vi "Teleop.vi"(10 "Match Info":T1={"Autonomous Elapsed Seconds"=0.0, "TeleOp Elapsed Seconds"=0.0, "Disabled Elapsed Seconds"=0.0, "Visited Autonomous"=FALSE, "Visited TeleOp"=FALSE, "Visited Disabled"=FALSE, "Autonomous Settings"={"Autonomous Style"=enum."Independent", "VI Refnum"=refnum}}, 11 "Call Context":T2) -> ()   [LabVIEW 2016]
doc: "This VI is called for each TeleOp packet received from the DS where the robot is not disabled. It is often used to read from the joysticks and update I/O or to update setpoints for timed control loops. It should complete and return within 20 milliseconds or it may miss DS packets."
uses:
  <vilib>/Rock Robotics/WPI/DriverStation/WPI_DriverStationDerivedRobotMode.ctl
  <vilib>/Rock Robotics/WPI/DriverStation/WPI_DriverStationMatch Info.ctl
  <vilib>/Rock Robotics/WPI/Solenoid/WPI_SolenoidValue.ctl
  <vilib>/Rock Robotics/WPI/Relay/WPI_RelayValue.ctl
  <vilib>/Rock Robotics/WPI/ThirdParty/CanMotor/TalonSRX/WPI_CANTalonSRX_BrakeOverride.ctl
  <vilib>/Rock Robotics/WPI/Utilities/WPI_GetSetVariantRefNum.vi
  <vilib>/Rock Robotics/Network Tables/NT Write Boolean Array.vi
  <vilib>/Rock Robotics/Network Tables/NT Write Numeric Array.vi
  <vilib>/Rock Robotics/Network Tables/NT Read Boolean.vi
  <vilib>/Rock Robotics/Network Tables/NT Read Number.vi
  <vilib>/Rock Robotics/WPI/Solenoid/WPI_SolenoidSetEnum.vi
  <vilib>/Rock Robotics/Network Tables/NT Write Boolean.vi
  <vilib>/Rock Robotics/WPI/RobotDrive/WPI_RobotDriveArcadeDrive_Standard(NoSaturation).vi
panel:
  out "Sample Slider 0":dbl(slide) scale=0.0..5.0
  out "Sample Boolean 1":bool
  out "Sample Boolean 0":bool
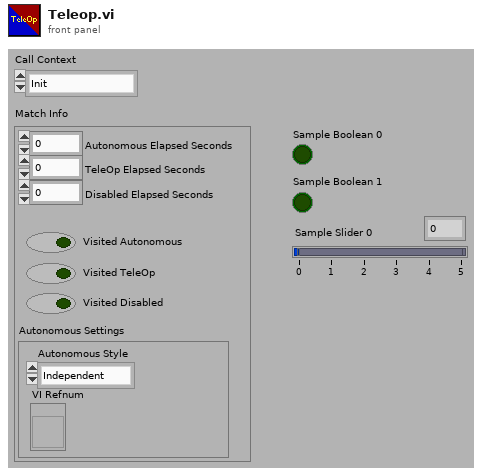
[diagram p1: front panel]
types:
  T1 = typedef "WPI_DriverStationMatch Info.ctl" = cluster{"Autonomous Elapsed Seconds":dbl, "TeleOp Elapsed Seconds":dbl, "Disabled Elapsed Seconds":dbl, "Visited Autonomous":bool, "Visited TeleOp":bool, "Visited Disabled":bool, "Autonomous Settings":cluster{"Autonomous Style":enum16{"Iterative", "Independent"}, "VI Refnum":refnum<vi>}}
  T2 = typedef "WPI_DriverStationDerivedRobotMode.ctl" = enum16{"Init", "Execute", "Stop"}
  T3 = typedef "WPI_CANTalonSRX_BrakeOverride.ctl" = enum8{"No Override", "Override to Coast", "Override to Brake"}
  T4 = typedef "WPI_SolenoidValue.ctl" = enum16{"Off", "On", "Forward", "Reverse"}
  T5 = typedef "WPI_RelayValue.ctl" = enum16{"Off", "On", "Forward", "Reverse"}
  T6 = typedef "WPI_JoystickDevRef.ctl" = cluster{"Device":T7}
  T7 = typedef "WPI_JoystickDeviceEnum.ctl" = enum16{"USB 0", "USB 1", "USB 2", "USB 3", "USB 4", "USB 5"}
  T8 = typedef "WPI_MotorControlDeviceRef.ctl" = cluster{"DeviceStatus":errorcluster, "Type":T9, "PWM":cluster{"PWM Channel":T10, "DeadBand":T11}, "CAN":cluster{"Device Number":u8, "SetOutput VI Ref":variant, "GetOutput VI Ref":variant, "Enable VI Ref":variant, "Disable VI Ref":variant, "Data":variant}, "Invert":bool}
  T9 = typedef "WPI_MotorControlType.ctl" = enum16{"PWM", "CAN"}
  T10 = typedef "FPGA_DIOPWMChannel.ctl" = enum8{"PWM 0", "PWM 1", "PWM 2", "PWM 3", "PWM 4", "PWM 5", "PWM 6", "PWM 7", "PWM 8", "PWM 9", "PWM MXP 0", "PWM MXP 1", "PWM MXP 2", "PWM MXP 3", "PWM MXP 4", "PWM MXP 5", "PWM MXP 6", "PWM MXP 7", "PWM MXP 8", "PWM MXP 9", "Invalid"}
  T11 = typedef "WPI_PWMDeadband.ctl" = cluster{"Name":string, "maxPositivePwm":i32, "minPositivePwm":i32, "centerPwm":i32, "maxNegativePwm":i32, "minNegativePwm":i32, "angularRange":u16}
  T12 = typedef "WPI_RobotDriveDevRef.ctl" = cluster{"DevStatus":errorcluster, "Motors[]":T8[], "Square Inputs":bool, "Max Output":dbl}
  T13 = typedef "WPI_RelayDevRef.ctl" = cluster{"DevStatus":errorcluster, "Relay Channel":T14, "Relay Direction":T15}
  T14 = typedef "FPGA_DIORelayChannel.ctl" = enum8{"Relay 0", "Relay 1", "Relay 2", "Relay 3", "Invalid"}
  T15 = typedef "WPI_RelayDirection.ctl" = enum16{"Both directions", "Forward only", "Reverse only"}
  T16 = typedef "WPI_SolenoidDevRef.ctl" = cluster{"DevStatus":errorcluster, "Pneumatics Control Module":u8, "Forward Solenoid Channel":T17, "Reverse Solenoid Channel":T17}
  T17 = typedef "WPI_SolenoidChannel.ctl" = enum8{"Solenoid 0", "Solenoid 1", "Solenoid 2", "Solenoid 3", "Solenoid 4", "Solenoid 5", "Solenoid 6", "Solenoid 7", "Invalid"}
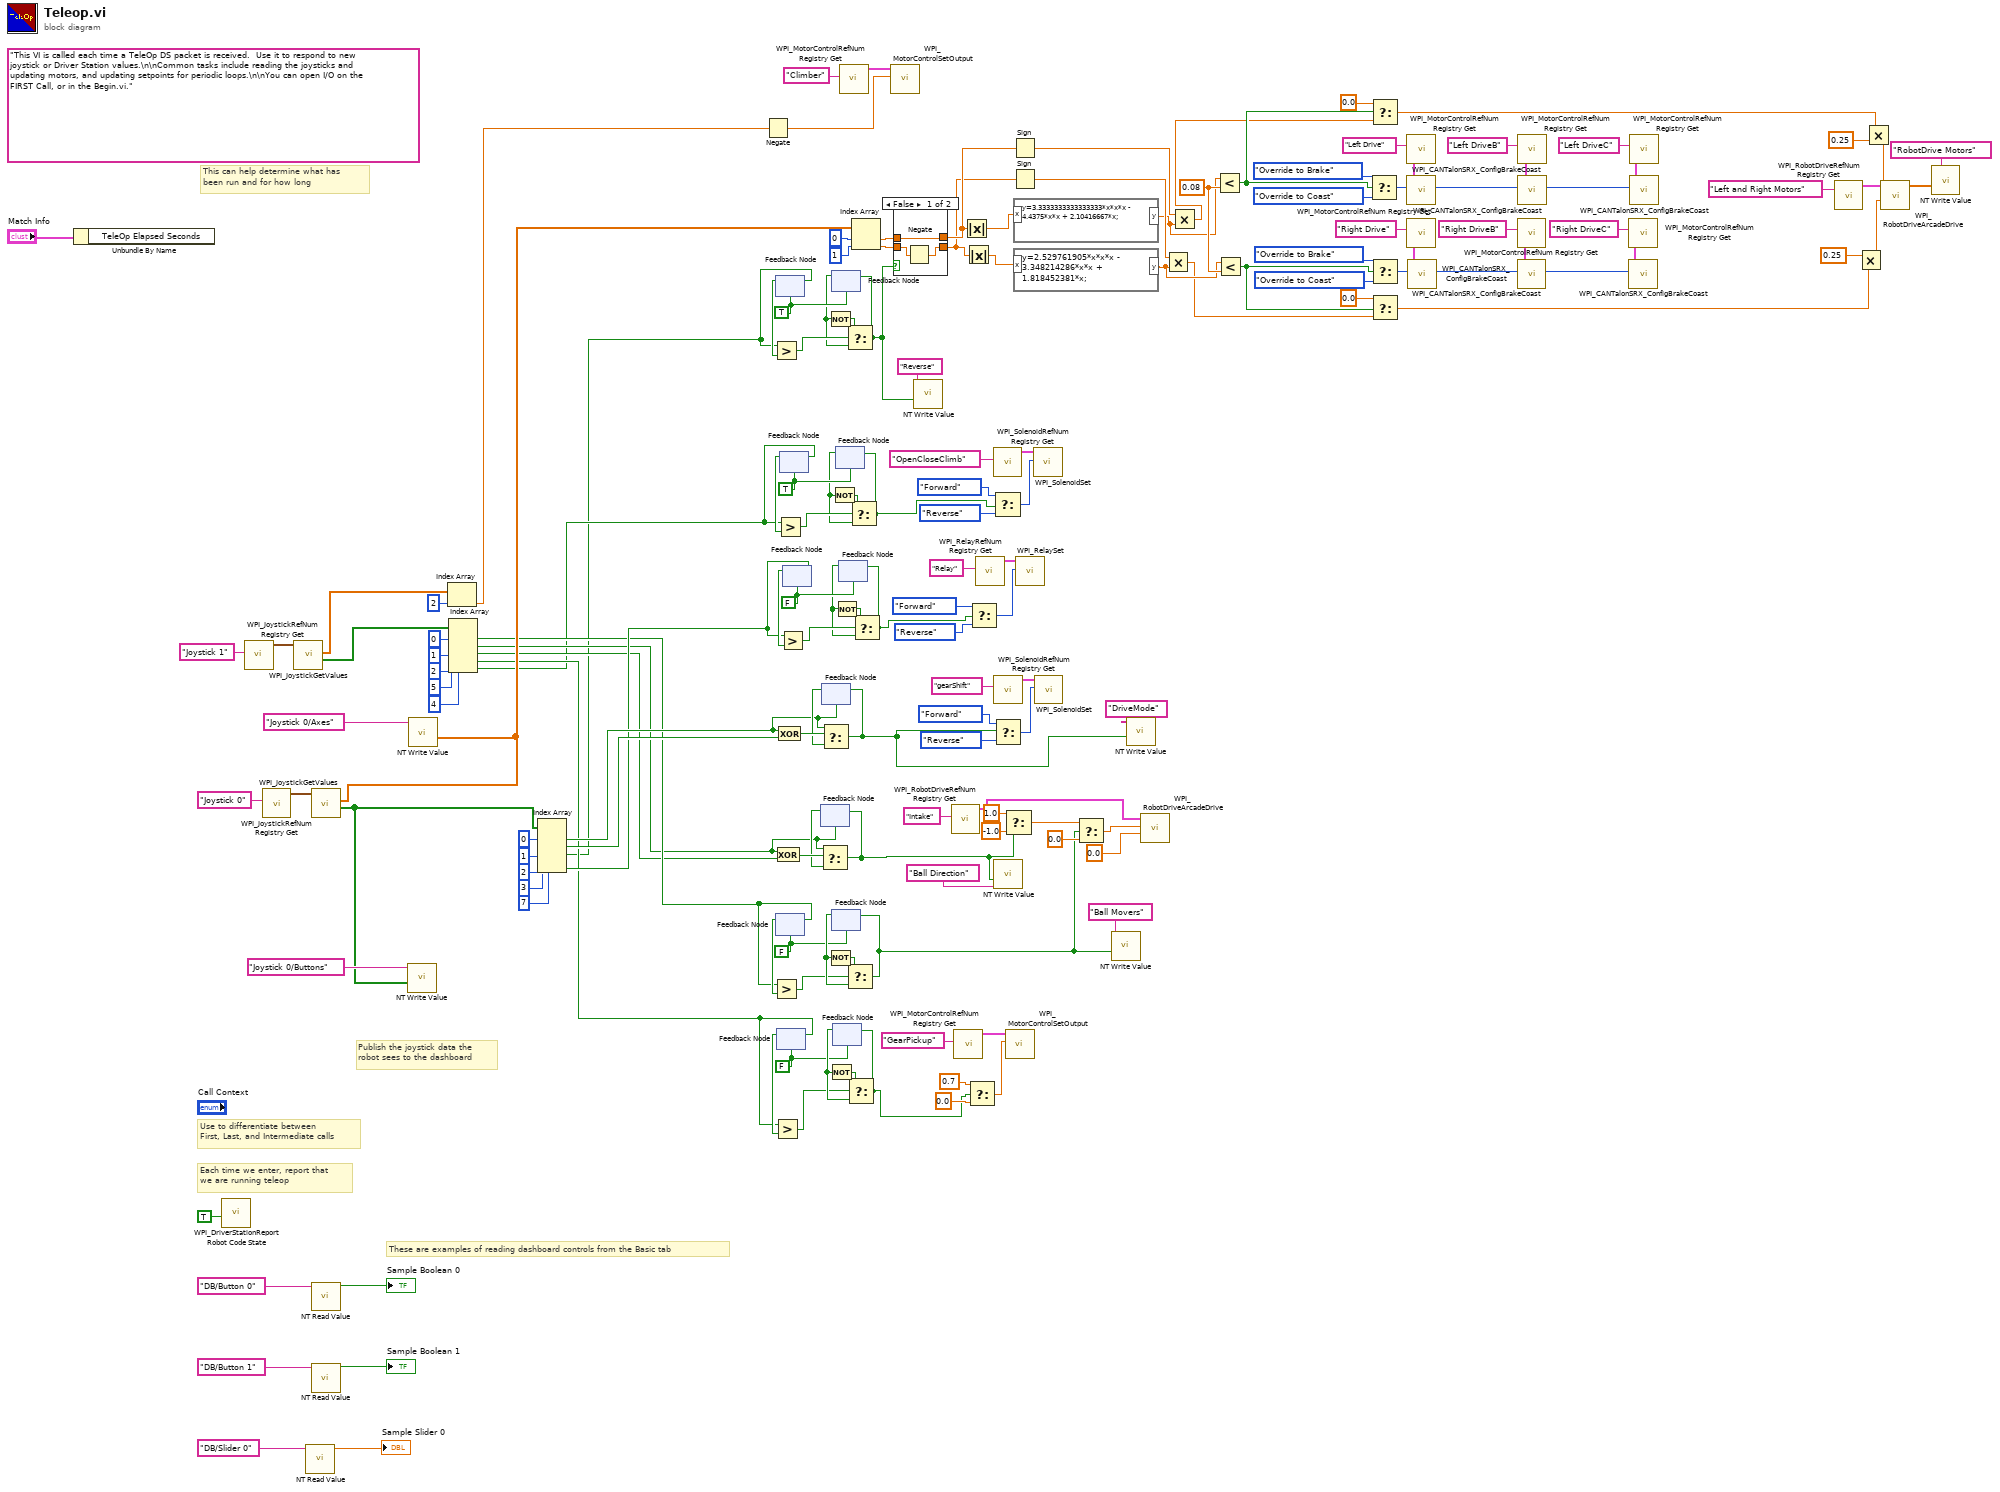
[diagram p0: block diagram]
diagram:
  w11 = TRUE ("Boolean")
  w67 = 0.08 ("y")
  w108 = FALSE ("Boolean")
  w133 = FALSE ("Boolean")
  w138 = FALSE ("Boolean")
  w143 = TRUE ("Boolean")
  (unwired) "This VI is called each time a TeleOp DS packet is received.  Use it to respond to new joystick or Driver Station values.\n\nCommon tasks include reading the joysticks and updating motors, and updating setpoints for periodic loops.\n\nYou can open I/O on the FIRST Call, or in the Begin.vi."
  # "These are examples of reading dashboard controls from the Basic tab"
  # "Publish the joystick data the\nrobot sees to the dashboard"
  # "Each time we enter, report that\nwe are running teleop"
  # "Use to differentiate between\nFirst, Last, and Intermediate calls"
  # "This can help determine what has\nbeen run and for how long"
  n1 = Unbundle By Name("Match Info") -> ()  [unwired: 1 out]
  n2 = call <vilib>:"WPI_DriverStationReport Robot Code State.vi"("TeleOp"=TRUE ("Autonomous")) -> ()  [unwired: 10 in, 1 out]
  n3 = call <vilib>:"WPI_JoystickRefNum Registry Get.vi"("refnum name"="Joystick 1") -> ("JoystickDevRef"=w45:T6)  [unwired: 1 in, 9 out]
  n4 = call <vilib>:"WPI_JoystickRefNum Registry Get.vi"("refnum name"="Joystick 0") -> ("JoystickDevRef"=w155:T6)  [unwired: 1 in, 9 out]
  n5 = call <vilib>:"WPI_JoystickGetValues.vi"("JoystickDevRef"=w45) -> ("Buttons"=w31:bool[], "Axes"=w17:dbl[])  [unwired: 6 in, 3 out]
  n6 = call-poly <vilib>:"NT Read Value.vi"("Name"="DB/Slider 0" ("refnum name")) -> ("Numeric"=→"Sample Slider 0":dbl)  [unwired: 9 in, 1 out]
  n7 = call <vilib>:"WPI_JoystickGetValues.vi"("JoystickDevRef"=w155) -> ("Buttons"=w38:bool[], "Axes"=w32:dbl[])  [unwired: 6 in, 3 out]
  n8 = call-poly <vilib>:"NT Read Value.vi"("Name"="DB/Button 0" ("refnum name")) -> ("Boolean"=→"Sample Boolean 0":bool)  [unwired: 9 in, 1 out]
  n9 = call-poly <vilib>:"NT Read Value.vi"("Name"="DB/Button 1" ("refnum name")) -> ("Boolean"=→"Sample Boolean 1":bool)  [unwired: 9 in, 1 out]
  n10 = call-poly <vilib>:"NT Write Value.vi"("Boolean Array"=w38, "Name"="Joystick 0/Buttons") -> ()  [unwired: 9 in, 1 out]
  n11 = call-poly <vilib>:"NT Write Value.vi"("Numeric Array"=w32, "Name"="Joystick 0/Axes") -> ()  [unwired: 9 in, 1 out]
  n12 = Index Array(array=w17, index=2) -> (element=w14:dbl)
  n13 = Index Array(array=w31, index #1=0 ("index"), index #2=1 ("index"), index #3=2 ("index"), index #4=5 ("index"), index #5=4 ("index")) -> (element #1=w29:bool, element #2=w25:bool, element #3=w26:bool, element #4=w21:bool, element #5=w18:bool)
  n14 = Index Array(array=w38, index #1=0 ("index"), index #2=1 ("index"), index #3=2 ("index"), index #4=3 ("index"), index #5=7 ("index")) -> (element #1=w36:bool, element #2=w37:bool, element #3=w7:bool, element #5=w33:bool)  [unwired: 1 out]
  n15 = Negate(x=w14) -> (-x=w5:dbl)
  n16 = Exclusive Or(1:w26, 2:w25) -> (0:w28:bool)
  n17 = Exclusive Or(1:w37, 2:w36) -> (0:w44:bool)
  n18 = feedback #1(w11) -> (w13:bool)
  n19 = Greater?(x=w7, y=w13) -> (0:w12:bool)
  n20 = feedback-in #1(w7) -> ()
  n21 = feedback #2(w108) -> (w106:bool)
  n22 = Greater?(x=w29, y=w106) -> (0:w107:bool)
  n23 = feedback-in #2(w29) -> ()
  n24 = feedback #3(w133) -> (w131:bool)
  n25 = Greater?(x=w21, y=w131) -> (0:w132:bool)
  n26 = feedback-in #3(w21) -> ()
  n27 = feedback #4(w143) -> (w145:bool)
  n28 = Greater?(x=w18, y=w145) -> (0:w144:bool)
  n29 = feedback-in #4(w18) -> ()
  n30 = feedback #5(w138) -> (w140:bool)
  n31 = Greater?(x=w33, y=w140) -> (0:w139:bool)
  n32 = feedback-in #5(w33) -> ()
  n33 = feedback #6(w25) -> (w27:bool)
  n34 = Select(t=w25, s=w28, f=w27) -> (s? t:f=w24:bool)
  n35 = feedback-in #6(w24) -> ()
  n36 = feedback #7(w36) -> (w43:bool)
  n37 = Select(t=w36, s=w44, f=w43) -> (s? t:f=w35:bool)
  n38 = feedback-in #7(w35) -> ()
  n39 = feedback #8(w11) -> (w10:bool)
  n40 = Not(x=w10) -> (.not. x?=w9:bool)
  n41 = feedback #9(w108) -> (w109:bool)
  n42 = Not(x=w109) -> (.not. x?=w110:bool)
  n43 = feedback #10(w133) -> (w134:bool)
  n44 = Not(x=w134) -> (.not. x?=w135:bool)
  n45 = feedback #11(w143) -> (w142:bool)
  n46 = Not(x=w142) -> (.not. x?=w141:bool)
  n47 = feedback #12(w138) -> (w137:bool)
  n48 = Not(x=w137) -> (.not. x?=w136:bool)
  n49 = call <vilib>:"WPI_MotorControlRefNum Registry Get.vi"("refnum name"="Climber") -> ("MotorControlDevRef"=w15:T8)  [unwired: 9 in, 1 out]
  n50 = Select(t=w9, s=w12, f=w10) -> (s? t:f=w8:bool)
  n51 = feedback-in #8(w8) -> ()
  n52 = Select(t=w110, s=w107, f=w109) -> (s? t:f=w91:bool)
  n53 = feedback-in #9(w91) -> ()
  n54 = Select(t=w135, s=w132, f=w134) -> (s? t:f=w95:bool)
  n55 = feedback-in #10(w95) -> ()
  n56 = Select(t=w141, s=w144, f=w142) -> (s? t:f=w130:bool)
  n57 = feedback-in #11(w130) -> ()
  n58 = Index Array(array=w32, index #1=0 ("index"), index #2=1 ("index")) -> (element #1=w84:dbl, element #2=w83:dbl)
  n59 = Select(t=w136, s=w139, f=w137) -> (s? t:f=w119:bool)
  n60 = feedback-in #12(w119) -> ()
  n61 = call <vilib>:"WPI_MotorControlSetOutput.vi"("Output"=w5, "MotorControlDevRef"=w15) -> ()  [unwired: 7 in, 3 out]
  n62 = case shown="False" w8 {
    tunnel: [w160 w161] -> w79
    tunnel: w84 -> [w160 w161]
    tunnel: [w158 w162] -> w78
    tunnel: w83 -> [w159 w162]
    frame False {
      n63 = Negate(x=w159) -> (-x=w158:dbl)
    }
    frame True {
    }
  }
  n64 = call-poly <vilib>:"NT Write Value.vi"("Boolean"=w8, "Name"="Reverse") -> ()  [unwired: 9 in, 1 out]
  n65 = call <vilib>:"WPI_RobotDriveRefNum Registry Get.vi"("refnum name"="Intake") -> ("RobotDriveDevRef"=w100:T12)  [unwired: 9 in, 1 out]
  n66 = call <vilib>:"WPI_MotorControlRefNum Registry Get.vi"("refnum name"="GearPickup") -> ("MotorControlDevRef"=w94:T8)  [unwired: 9 in, 1 out]
  n67 = Absolute Value(x=w79) -> (abs(x)=w81:dbl)
  n68 = Absolute Value(x=w78) -> (abs(x)=w80:dbl)
  n69 = Select(t=0.7, s=w95, f=0.0 ("Output")) -> (s? t:f=w96:dbl)
  n70 = Select(t=WPI_RelayValue."Forward" ("RelayValue"), s=w119, f=WPI_RelayValue."Reverse") -> (s? t:f=w122:T5)
  n71 = call <vilib>:"WPI_RelayRefNum Registry Get.vi"("refnum name"="Relay") -> ("RelayDevRef"=w123:T13)  [unwired: 9 in, 1 out]
  n72 = call <vilib>:"WPI_SolenoidRefNum Registry Get.vi"("refnum name"="OpenCloseClimb") -> ("SolenoidDevRef"=w126:T16)  [unwired: 9 in, 1 out]
  n73 = Select(t=WPI_SolenoidValue."Forward" ("Value"), s=w130, f=WPI_SolenoidValue."Reverse" ("Value")) -> (s? t:f=w125:T4)
  n74 = call <vilib>:"WPI_SolenoidRefNum Registry Get.vi"("refnum name"="gearShift") -> ("SolenoidDevRef"=w114:T16)  [unwired: 9 in, 1 out]
  n75 = Select(t=WPI_SolenoidValue."Forward" ("Value"), s=w35, f=WPI_SolenoidValue."Reverse" ("Value")) -> (s? t:f=w116:T4)
  n76 = call-poly <vilib>:"NT Write Value.vi"("Boolean"=w24, "Name"="Ball Direction") -> ()  [unwired: 9 in, 1 out]
  n77 = Select(t=1.0, s=w24, f=-1.0) -> (s? t:f=w104:dbl)
  n78 = call <vilib>:"WPI_MotorControlSetOutput.vi"("Output"=w96, "MotorControlDevRef"=w94) -> ()  [unwired: 7 in, 3 out]
  n79 = Sign(1:w79) -> (0:w76:dbl)
  n80 = Sign(1:w78) -> (0:w77:dbl)
  n81 = formula code="y=3.3333333333333333*x*x*x - 4.4375*x*x + 2.10416667*x;"("x"=w81) -> ("y"=w63:dbl)
  n82 = formula code="y=2.529761905*x*x*x - 3.348214286*x*x + 1.818452381*x;"("x"=w80) -> ("y"=w61:dbl)
  n83 = call <vilib>:"WPI_RelaySet.vi"("RelayValue"=w122, "RelayDevRef"=w123) -> ()  [unwired: 8 in, 2 out]
  n84 = call-poly <vilib>:"WPI_SolenoidSet.vi"("Value"=w125, "SolenoidDevRef"=w126) -> ()  [unwired: 8 in, 2 out]
  n85 = call-poly <vilib>:"WPI_SolenoidSet.vi"("Value"=w116, "SolenoidDevRef"=w114) -> ()  [unwired: 8 in, 2 out]
  n86 = Select(t=w104, s=w91, f=0.0) -> (s? t:f=w103:dbl)
  n87 = call-poly <vilib>:"NT Write Value.vi"("Boolean"=w91, "Name"="Ball Movers") -> ()  [unwired: 9 in, 1 out]
  n88 = call-poly <vilib>:"NT Write Value.vi"("Boolean"=w35, "Name"="DriveMode") -> ()  [unwired: 9 in, 1 out]
  n89 = call-poly <vilib>:"WPI_RobotDriveArcadeDrive.vi"("Y axis value"=0.0, "X axis value"=w103, "RobotDriveDevRef"=w100) -> ()  [unwired: 6 in, 3 out]
  n90 = Multiply(x=w77, y=w61) -> (x*y=w60:dbl)
  n91 = Multiply(x=w76, y=w63) -> (x*y=w62:dbl)
  n92 = Less?(x=w63, y=w67) -> (x < y?=w65:bool)
  n93 = Less?(x=w61, y=w67) -> (x < y?=w66:bool)
  n94 = Select(t=WPI_CANTalonSRX_BrakeOverride."Override to Brake" ("Brake / Coast Mode"), s=w65, f=WPI_CANTalonSRX_BrakeOverride."Override to Coast") -> (s? t:f=w50:T3)
  n95 = Select(t=0.0, s=w65, f=w62) -> (s? t:f=w49:dbl)
  n96 = Select(t=WPI_CANTalonSRX_BrakeOverride."Override to Brake" ("Brake / Coast Mode"), s=w66, f=WPI_CANTalonSRX_BrakeOverride."Override to Coast") -> (s? t:f=w55:T3)
  n97 = Select(t=0.0, s=w66, f=w60) -> (s? t:f=w48:dbl)
  n98 = call <vilib>:"WPI_MotorControlRefNum Registry Get.vi"("refnum name"="Left Drive") -> ("MotorControlDevRef"=w68:T8)  [unwired: 9 in, 1 out]
  n99 = call <vilib>:"WPI_CANTalonSRX_ConfigBrakeCoast.vi"("Brake / Coast Mode"=w50, "CAN Talon SRX Ref"=w68) -> ()  [unwired: 8 in, 2 out]
  n100 = call <vilib>:"WPI_MotorControlRefNum Registry Get.vi"("refnum name"="Right Drive") -> ("MotorControlDevRef"=w71:T8)  [unwired: 9 in, 1 out]
  n101 = call <vilib>:"WPI_CANTalonSRX_ConfigBrakeCoast.vi"("Brake / Coast Mode"=w55, "CAN Talon SRX Ref"=w71) -> ()  [unwired: 8 in, 2 out]
  n102 = call <vilib>:"WPI_MotorControlRefNum Registry Get.vi"("refnum name"="Right DriveB") -> ("MotorControlDevRef"=w58:T8)  [unwired: 9 in, 1 out]
  n103 = call <vilib>:"WPI_CANTalonSRX_ConfigBrakeCoast.vi"("Brake / Coast Mode"=w55, "CAN Talon SRX Ref"=w58) -> ()  [unwired: 8 in, 2 out]
  n104 = call <vilib>:"WPI_MotorControlRefNum Registry Get.vi"("refnum name"="Left DriveB") -> ("MotorControlDevRef"=w53:T8)  [unwired: 9 in, 1 out]
  n105 = call <vilib>:"WPI_CANTalonSRX_ConfigBrakeCoast.vi"("Brake / Coast Mode"=w50, "CAN Talon SRX Ref"=w53) -> ()  [unwired: 8 in, 2 out]
  n106 = call <vilib>:"WPI_MotorControlRefNum Registry Get.vi"("refnum name"="Right DriveC") -> ("MotorControlDevRef"=w56:T8)  [unwired: 9 in, 1 out]
  n107 = call <vilib>:"WPI_CANTalonSRX_ConfigBrakeCoast.vi"("Brake / Coast Mode"=w55, "CAN Talon SRX Ref"=w56) -> ()  [unwired: 8 in, 2 out]
  n108 = call <vilib>:"WPI_MotorControlRefNum Registry Get.vi"("refnum name"="Left DriveC") -> ("MotorControlDevRef"=w51:T8)  [unwired: 9 in, 1 out]
  n109 = call <vilib>:"WPI_CANTalonSRX_ConfigBrakeCoast.vi"("Brake / Coast Mode"=w50, "CAN Talon SRX Ref"=w51) -> ()  [unwired: 8 in, 2 out]
  n110 = call <vilib>:"WPI_RobotDriveRefNum Registry Get.vi"("refnum name"="Left and Right Motors") -> ("RobotDriveDevRef"=w89:T12)  [unwired: 1 in, 9 out]
  n111 = Multiply(x=0.25, y=w48) -> (x*y=w4:dbl)
  n112 = Multiply(x=w49, y=0.25) -> (x*y=w3:dbl)
  n113 = call-poly <vilib>:"WPI_RobotDriveArcadeDrive.vi"("Y axis value"=w4, "X axis value"=w3, "RobotDriveDevRef"=w89) -> ("Motor Values"=w88:dbl[])  [unwired: 6 in, 2 out]
  n114 = call-poly <vilib>:"NT Write Value.vi"("Numeric Array"=w88, "Name"="RobotDrive Motors") -> ()  [unwired: 9 in, 1 out]
